vi "Generate Key.vi"(11 "ID":string) -> (3 "Key":string)   [LabVIEW 2020, in "Data Viewer.lvlib"]
uses:
  Data Viewer.lvlib
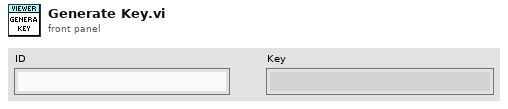
[diagram p1: front panel]
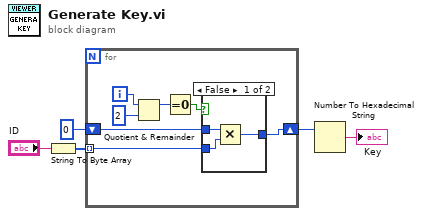
[diagram p0: block diagram]
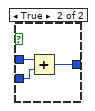
[diagram p2: hidden frame]
diagram:
  n1 = String To Byte Array(string="ID") -> (unsigned byte array=w3:u8[])
  n2 = for {
    tunnel: w3 -> [w6] mode=indexing
    shift-right: [w11] -> w4
    shift-left: u32 0 -> [w12]
    i -> [w10]
    n3 = Quotient & Remainder(x=w10, y=2) -> (x-y*floor(x/y)=w8:i32)  [unwired: 1 out]
    n4 = Equal To 0?(x=w8) -> (x = 0?=w7:bool)
    n5 = case shown="False" w7 {
      tunnel: w12 -> [w13 w18]
      tunnel: [w15 w17] -> w11
      tunnel: w6 -> [w14 w16]
      frame False {
        n6 = Multiply(x=w13, y=w14) -> (x*y=w15:u32)
      }
      frame True {
        n7 = Add(x=w18, y=w16) -> (x+y=w17:u32)
      }
    }
  }
  n8 = Number To Hexadecimal String(2:w4) -> (0:→"Key":string)  [unwired: 1 in]
